vi "Add Tx Label.vi"(4 "scheduled transmit period (us)":u32=1000, 6 "transfer type":T2, 7 "label (Display)":u32, 8 "error in":errorcluster, 9 "SDI value":T3=-1 items=["All"=-1, "0 (b00)"=0, "1 (b01)"=1, "2 (b10)"=2, "3 (b11)"=3], 10 "label (Dec)":u32, 11 "port in":T1 format="%.0x") -> (0 "error out":errorcluster, 2 "label":T1 format="%.0x", 3 "port out":T1 format="%.0x")   [LabVIEW 2020, in "Ballard ARINC 429 Scripting.lvlib"]
doc: "Adds a Tx label to the specified outgoing (Tx) port. Returns the newly added <b>label</b> reference."
uses:
  Ballard ARINC 429 Scripting.lvlib
  Constants.vi
  ARINC 429/ARINC 429 Scripting.lvlib
  <vilib>/NI VeriStand/Custom Device API/Custom Device Channel Type.ctl
  <vilib>/NI VeriStand/Custom Device API/Custom Device API.lvlib
  <vilib>/NI VeriStand/Custom Device API/Custom Device Channel.ctl
  Shared/Label Properties.ctl
  Shared/Label.ctl
  Import/ARINC 429 Import.lvlib
  <vilib>/NI VeriStand/Custom Device API/Custom Device Item Ref.ctl
  <vilib>/NI VeriStand/Custom Device Offline API/Custom Device Offline API.lvlib
  Shared/Transfer Type.ctl
  Shared/SDI.ctl
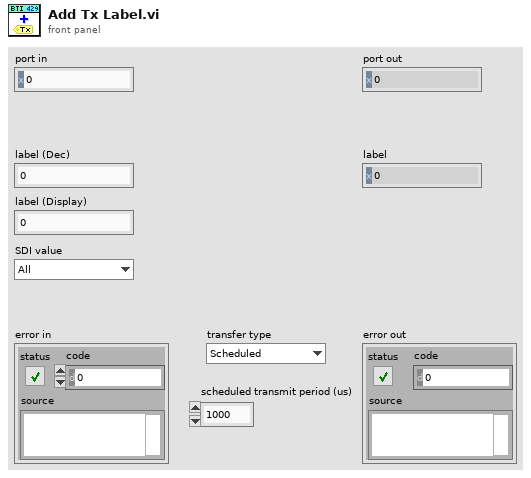
[diagram p1: front panel]
types:
  T1 = typedef "Custom Device API.lvlib/Custom Device Item Ref.ctl" = u64
  T2 = typedef "Transfer Type.ctl" = enum16{"Scheduled", "Acyclic", "Block", "Strobe"}
  T3 = typedef "SDI.ctl" = i32
  T4 = typedef "Direction.ctl" = enum16{"Rx", "Tx"}
  T5 = typedef "Custom Device API.lvlib/Custom Device Channel.ctl" = cluster{"Type":T6, "Units":string, "Default Value":dbl, "Faultable":bool, "Scalable":bool}
  T6 = typedef "Custom Device API.lvlib/Custom Device Channel Type.ctl" = enum16{"Input", "Output"}
  T7 = typedef "Label Properties.ctl" = cluster{"label (Dec)":T8, "SDI value":u8, "SDI enabled":bool}
  T8 = typedef "Label.ctl" = u8
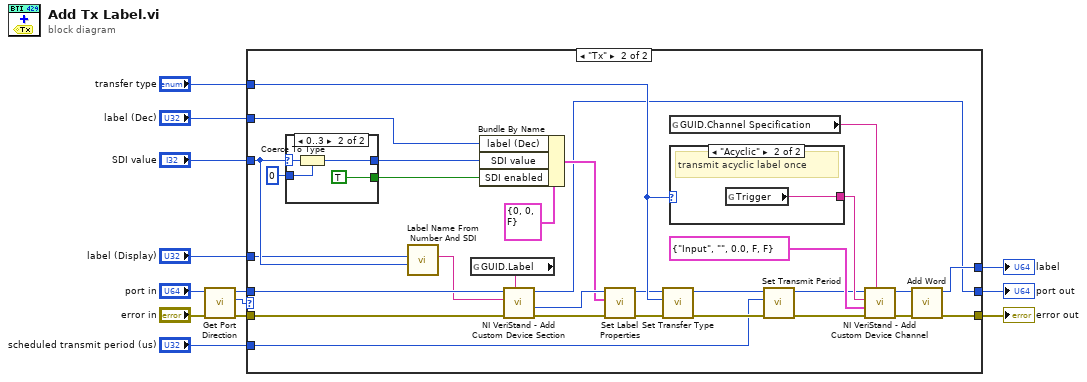
[diagram p0: block diagram]
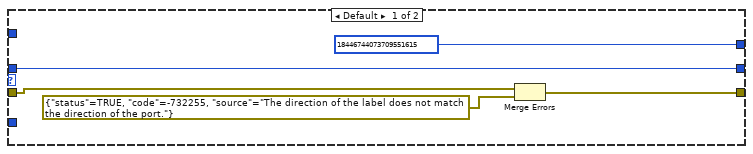
[diagram p2: hidden frame]
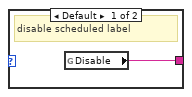
[diagram p3: hidden frame]
diagram:
  n1 = call "Get Port Direction.vi"("error in"="error in", "port ref in"="port in") -> ("error out"=w9:errorcluster, "direction"=w3:T4, "port ref out"=w10:T1)  [unwired: 7 in]
  n2 = case shown="\"Tx\"" w3 {
    tunnel: [w15 w41] -> w13
    tunnel: w10 -> [w18 w38]
    tunnel: w9 -> [w16 w37]
    tunnel: [T1 18446744073709551615 ("label ref out") w34] -> w8
    tunnel: [w18 w24] -> w7
    tunnel: "transfer type" -> [_ w33]
    tunnel: "label (Dec)" -> [_ w30]
    tunnel: "SDI value" -> [_ w28]
    tunnel: "scheduled transmit period (us)" -> [_ w20]
    tunnel: "label (Display)" -> [_ w19]
    frame Default {
      n3 = Merge Errors(w16, errorcluster {"status"=TRUE, "code"=-732255, "source"="The direction of the label does not match the direction of the port."} ("error in")) -> (w15:errorcluster)
    }
    frame "Tx" {
      n4 = case shown="0..3" w28 {
        selector: w28 -> [_ w55]
        tunnel: [w51 w52] -> w29
        tunnel: u8 0 ("SDI value") -> [w51 w54]
        tunnel: [_ TRUE] -> w35
        frame Default {
        }
        frame 0..3 {
          n5 = Coerce To Type(0:w55, 1:w54) -> (2:w52:u8)
        }
      }
      n6 = call "Label Name From Number And SDI.vi"("SDI value"=w28, "label (Display)"=w19) -> ("label name"=w31:string)  [unwired: 9 in]
      n7 = global read "Constants.vi" "GUID.Label"() -> (w42:string)
      n8 = Bundle By Name(cluster=T7 {"label (Dec)"=0, "SDI value"=0, "SDI enabled"=FALSE} ("label properties"), "label (Dec)"=w30, "SDI value"=w29, "SDI enabled"=w35) -> (w39:T7)
      n9 = call <vilib>:"NI VeriStand - Add Custom Device Section.vi"("GUID (Default Section)"=w42, "error in (no error)"=w37, "Section Name"=w31, "Parent Ref in"=w38) -> ("error out"=w44:errorcluster, "Section Ptr"=w43:T1, "Parent Ref out"=w24:T1)  [unwired: 4 in, 1 out]
      n10 = call "Set Label Properties.vi"("error in"=w44, "label properties"=w39, "label ref"=w43) -> ("error out"=w45:errorcluster, "label ref out"=w32:T1)  [unwired: 7 in]
      n11 = call "Set Transfer Type.vi"("error in"=w45, "transfer type"=w33, "label ref in"=w32) -> ("error out"=w46:errorcluster, "label ref out"=w22:T1)  [unwired: 7 in]
      n12 = global read "Constants.vi" "GUID.Channel Specification"() -> (w27:string)
      n13 = case shown="\"Acyclic\"" w33 {
        tunnel: [w49 w50] -> w26
        frame Default {
          # "disable scheduled label"
          n14 = global read "Constants.vi" "Disable"() -> (w49:string)
        }
        frame "Acyclic" {
          # "transmit acyclic label once"
          n15 = global read "Constants.vi" "Trigger"() -> (w50:string)
        }
      }
      n16 = call "Set Transmit Period.vi"("error in"=w46, "transmit period (us)"=w20, "label ref"=w22) -> ("error out"=w23:errorcluster, "label ref out"=w21:T1)  [unwired: 7 in]
      n17 = call <vilib>:"NI VeriStand - Add Custom Device Channel.vi"("GUID (Default Channel)"=w27, "error in (no error)"=w23, "Channel"=T5 {"Type"=enum."Input", "Units"="", "Default Value"=0.0, "Faultable"=FALSE, "Scalable"=FALSE}, "Channel Name"=w26, "Parent Ref in"=w21) -> ("error out"=w47:errorcluster, "Parent Ref out"=w48:T1)  [unwired: 3 in, 2 out]
      n18 = call "Add Word.vi"("error in"=w47, "label ref"=w48) -> ("error out"=w41:errorcluster, "label ref out"=w34:T1)  [unwired: 6 in, 2 out]
    }
  }
  "label" <- w8
  "error out" <- w13
  "port out" <- w7
